vi "DialogCreateClass_ReadTemplatesFilterSettings.vi"(11 "ProviderShortName":string) -> (2 "TemplateFilter":T1, 3 "Section":string)   [LabVIEW 2020, in "ClassWriterNative.lvclass"]
uses:
  <resource>/Framework/Providers/Open_GDS/ClassProviders/Provider_LvNativeClass/ClassWriterNative_class/ClassWriterNative.lvclass
  <vilib>/Utility/config.llb/Read Key (String).vi
  <vilib>/Utility/config.llb/NI_LVConfig.lvlib
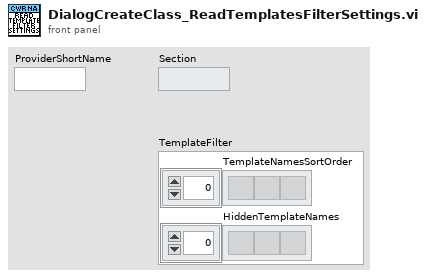
[diagram p1: front panel]
types:
  T1 = cluster{"TemplateNamesSortOrder":string[], "HiddenTemplateNames":string[]}
  T2 = typedef "NI_LVConfig.lvlib/Config Data RefNum.ctl" = refnum<k1>
  T3 = cluster{"Split String":string[], "Split String":string[]}
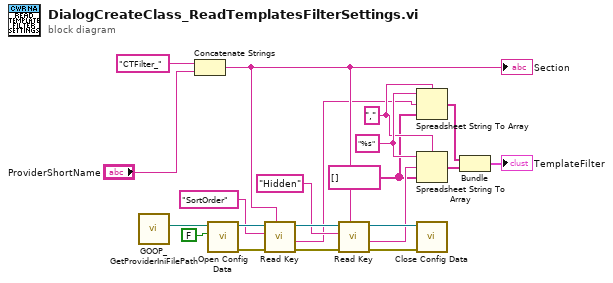
[diagram p0: block diagram]
diagram:
  w4 = "," ("Split Pattern")
  w5 = "%s" ("format string")
  w3 = string[] [] ("Split String")
  n1 = call <resource>:"GOOP_GetProviderIniFilePath.vi"() -> ("ProviderIniPath"=w17:path)  [unwired: 10 in, 1 out]
  n2 = Concatenate Strings("CTFilter_" ("regular expression (\"\")"), "ProviderShortName") -> (w12:string)
  "Section" <- w12
  n3 = call <vilib>:"Open Config Data.vi"("create file if necessary (T)"=FALSE, "configuration file path"=w17) -> ("error out"=w20:errorcluster, "refnum"=w19:T2)  [unwired: 7 in, 1 out]
  n4 = call-poly <vilib>:"Read Key.vi"("section"=w12, "error in (no error)"=w20, "key"="SortOrder", "refnum"=w19) -> ("error out"=w8:errorcluster, "value"=w2:string, "refnum out"=w14:T2)  [unwired: 4 in, 1 out]
  n5 = call-poly <vilib>:"Read Key.vi"("section"=w12, "error in (no error)"=w8, "key"="Hidden", "refnum"=w14) -> ("error out"=w9:errorcluster, "value"=w7:string, "refnum out"=w13:T2)  [unwired: 4 in, 1 out]
  n6 = Spreadsheet String To Array(delimiter (Tab)=w4, format string=w5, spreadsheet string=w2, array type (2D Dbl)=w3) -> (array=w1:string[])
  n7 = Spreadsheet String To Array(delimiter (Tab)=w4, format string=w5, spreadsheet string=w7, array type (2D Dbl)=w3) -> (array=w6:string[])
  n8 = call <vilib>:"Close Config Data.vi"("error in (no error)"=w9, "refnum"=w13) -> ()  [unwired: 8 in, 2 out]
  n9 = Bundle("Split String"=w1, "Split String"=w6) -> (→"TemplateFilter":T3)  [unwired: 1 in]
